vi "[ce] Index Range to-from DBL.vi"(10 "Index Range":cluster{"Initial index":i32, "Final index":i32}, 11 "dbl scalar":dbl) -> (2 "dbl scalar out":dbl, 3 "Index Range out":cluster{"Initial index":i32, "Final index":i32})   [LabVIEW 2021]
doc: "::: CalcExpress Toolkit :::\nCopyright (c) 2000-2026 Konstantin Shifershteyn. All rights reserved."
uses:
  cersrc/celveng32.dll
panel:
  # ":"
  # ":"
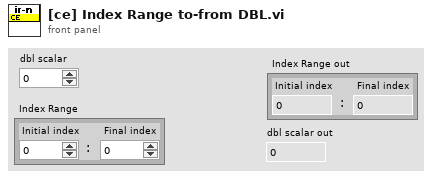
[diagram p1: front panel]
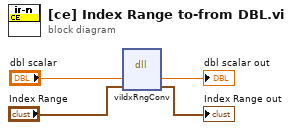
[diagram p0: block diagram]
diagram:
  n1 = dll-call lib="C:/LV Projects/CalcExpress 40 LV2021/vi.lib/addons/CalcExpress/cersrc/celveng*.dll" fn="viIdxRngConv"("n"="dbl scalar", "ir"="Index Range") -> ("n"=→"dbl scalar out":dbl, "ir"=→"Index Range out":cluster{"Initial index":i32, "Final index":i32})  [unwired: 4 in, 2 out]
